vi "PS Chart.vi"(7 "all?":bool, 8 "error in (no error)":errorcluster, 10 "Power Spectrum / PSD":cluster{"f0":dbl, "df":dbl, "magnitude":dbl[]}[](array[cluster]), 11 "WFGraph (WDT) in":refnum<vi>) -> (0 "error out":errorcluster, 3 "Chart":dbl[][](array[numeric]))   [LabVIEW 2019, in "Instrument.Lockin.lvlib" / "Instrument UI.Lockin.lvclass"]
uses:
  Instrument UI.Lockin.lvclass
  <vilib>/Waveform/WDTOps.llb/WDT Waveform to XY Pairs DBL.vi
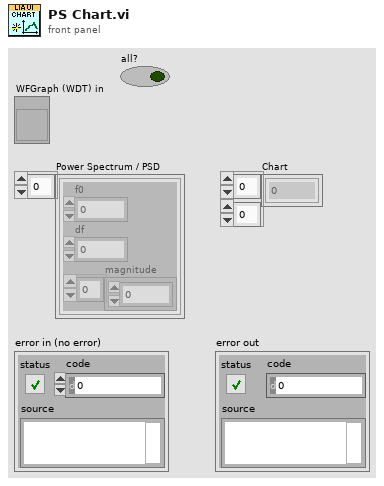
[diagram p1: front panel]
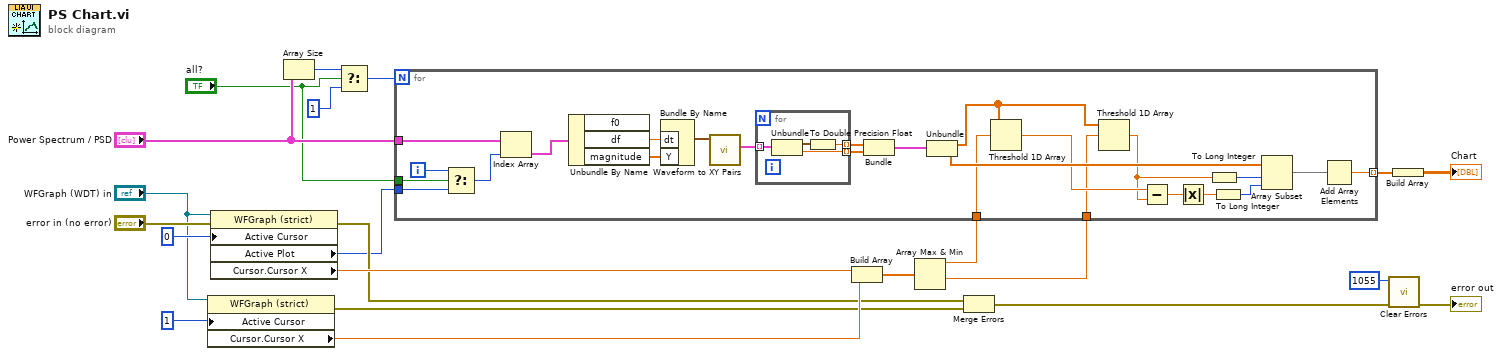
[diagram p0: block diagram]
diagram:
  n1 = property on="Property Node" class="WFGraph (strict)"(reference="WFGraph (WDT) in", "Active Cursor"=u32 1) -> (error out=w17:errorcluster, "Cursor.Cursor X"=w21:dbl)  [unwired: 1 in, 1 out]
  n2 = property on="Property Node" class="WFGraph (strict)"(reference="WFGraph (WDT) in", error in="error in (no error)", "Active Cursor"=u32 0) -> (error out=w8:errorcluster, "Active Plot"=w3:u32, "Cursor.Cursor X"=w12:dbl)  [unwired: 1 out]
  n3 = Array Size(array="Power Spectrum / PSD") -> (size(s)=w5:i32)
  n4 = Select(t=w5, s="all?", f=1) -> (s? t:f=w6:i32)
  n5 = Build Array(w12, w21) -> (w13:dbl[])
  n6 = Array Max & Min(array=w13) -> (max value=w7:dbl, min value=w10:dbl)  [unwired: 2 out]
  n7 = for {
    N: w6 -> [_]
    tunnel: [w47] -> w18 mode=indexing
    tunnel: "Power Spectrum / PSD" -> [w39]
    tunnel: w10 -> [w32]
    tunnel: w7 -> [w30]
    tunnel: w3 -> [w24]
    tunnel: "all?" -> [w23]
    i -> [w26]
    n8 = Select(t=w26, s=w23, f=w24) -> (s? t:f=w25:u32)
    n9 = Index Array(array=w39, index=w25) -> (element=w38:cluster{"f0":dbl, "df":dbl, "magnitude":dbl[]})
    n10 = Unbundle By Name(w38) -> ("df"=w45:dbl, "magnitude"=w44:dbl[])  [unwired: 1 out]
    n11 = Bundle By Name("dt"=w45, "Y"=w44) -> (w43:waveform(dbl))  [unwired: 1 in]
    n12 = call-poly <vilib>:"Waveform to XY Pairs.vi"("waveform in"=w43) -> ("XY pairs"=w42:cluster{"x":timestamp, "y":dbl}[])  [unwired: 8 in, 2 out]
    n13 = for {
      tunnel: w42 -> [w51] mode=indexing
      tunnel: [w49] -> w40 mode=indexing
      tunnel: [w48] -> w41 mode=indexing
      n14 = Unbundle(w51) -> ("x"=w50:timestamp, "y"=w49:dbl)
      n15 = To Double Precision Float(number=w50) -> (double precision float=w48:dbl)
    }
    n16 = Bundle(w41, w40) -> (w46:cluster{dbl[], dbl[]})  [unwired: 1 in]
    n17 = Unbundle(w46) -> (w31:dbl[], w37:dbl[])
    n18 = Threshold 1D Array(2:w30, 3:w31) -> (0:w36:dbl)  [unwired: 1 in]
    n19 = Threshold 1D Array(2:w32, 3:w31) -> (0:w33:dbl)  [unwired: 1 in]
    n20 = Subtract(x=w36, y=w33) -> (x-y=w34:dbl)
    n21 = Absolute Value(x=w34) -> (abs(x)=w27:dbl)
    n22 = To Long Integer(number=w33) -> (32bit integer=w29:i32)
    n23 = To Long Integer(number=w27) -> (32bit integer=w28:i32)
    n24 = Array Subset(array=w37, index=w29, length=w28) -> (w35:dbl[])
    n25 = Add Array Elements(numeric array=w35) -> (sum=w47:dbl)
  }
  n26 = Merge Errors(w8, w17) -> (w14:errorcluster)
  n27 = call <vilib>:"Clear Errors.vi"("error in (no error)"=w14, "specific error code to clear (0: all)"=1055) -> ("error out"=→"error out":errorcluster)  [unwired: 4 in, 1 out]
  n28 = Build Array(w18) -> (→"Chart":dbl[][])
